vi "Backpressure test CIF Pcap.vi"() -> ()   [LabVIEW 2021]
uses:
  Iceoryx.lvlib
  typedef/CIF Pcap Publisher Configuration.ctl
  typedef/CIF Pcap Subscriber Configuration.ctl
  typedef/CIF Channel Header Publisher.ctl
panel:
  out "status":string
  out "pass":bool
  out "error out":errorcluster
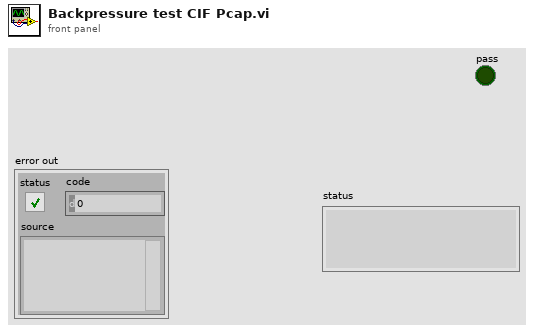
[diagram p1: front panel]
types:
  T1 = typedef "Iceoryx.lvlib/CIF Pcap Subscriber Configuration.ctl" = cluster{"Name":string, "Topic":string, "Link Type":u32, "Backpressure":bool}
  T2 = typedef "Iceoryx.lvlib/CIF Pcap Publisher Configuration.ctl" = cluster{"Name":string, "Topic":string, "Link Type":u32, "Descriptor":string, "Max Bytes":u32, "Best Effort Subscribers":u32, "Backpressure Subscribers":u32, "Best Effort Queue Depth":u32, "Backpressure Queue Depth":u32}
  T3 = typedef "Iceoryx.lvlib/CIF Channel Header Publisher.ctl" = cluster{"T0":i64, "T_Out":i64, "T_Tx":i64, "ClockID":u8}
  T4 = typedef "Iceoryx.lvlib/CIF Publisher Refnum.ctl" = cluster{"refnum":u64, "CIF Pub":enum8{"cifpub"}}
  T5 = typedef "Iceoryx.lvlib/CIF Subscriber Refnum.ctl" = cluster{"refnum":u64, "CIF Sub":enum8{"cifsub"}}
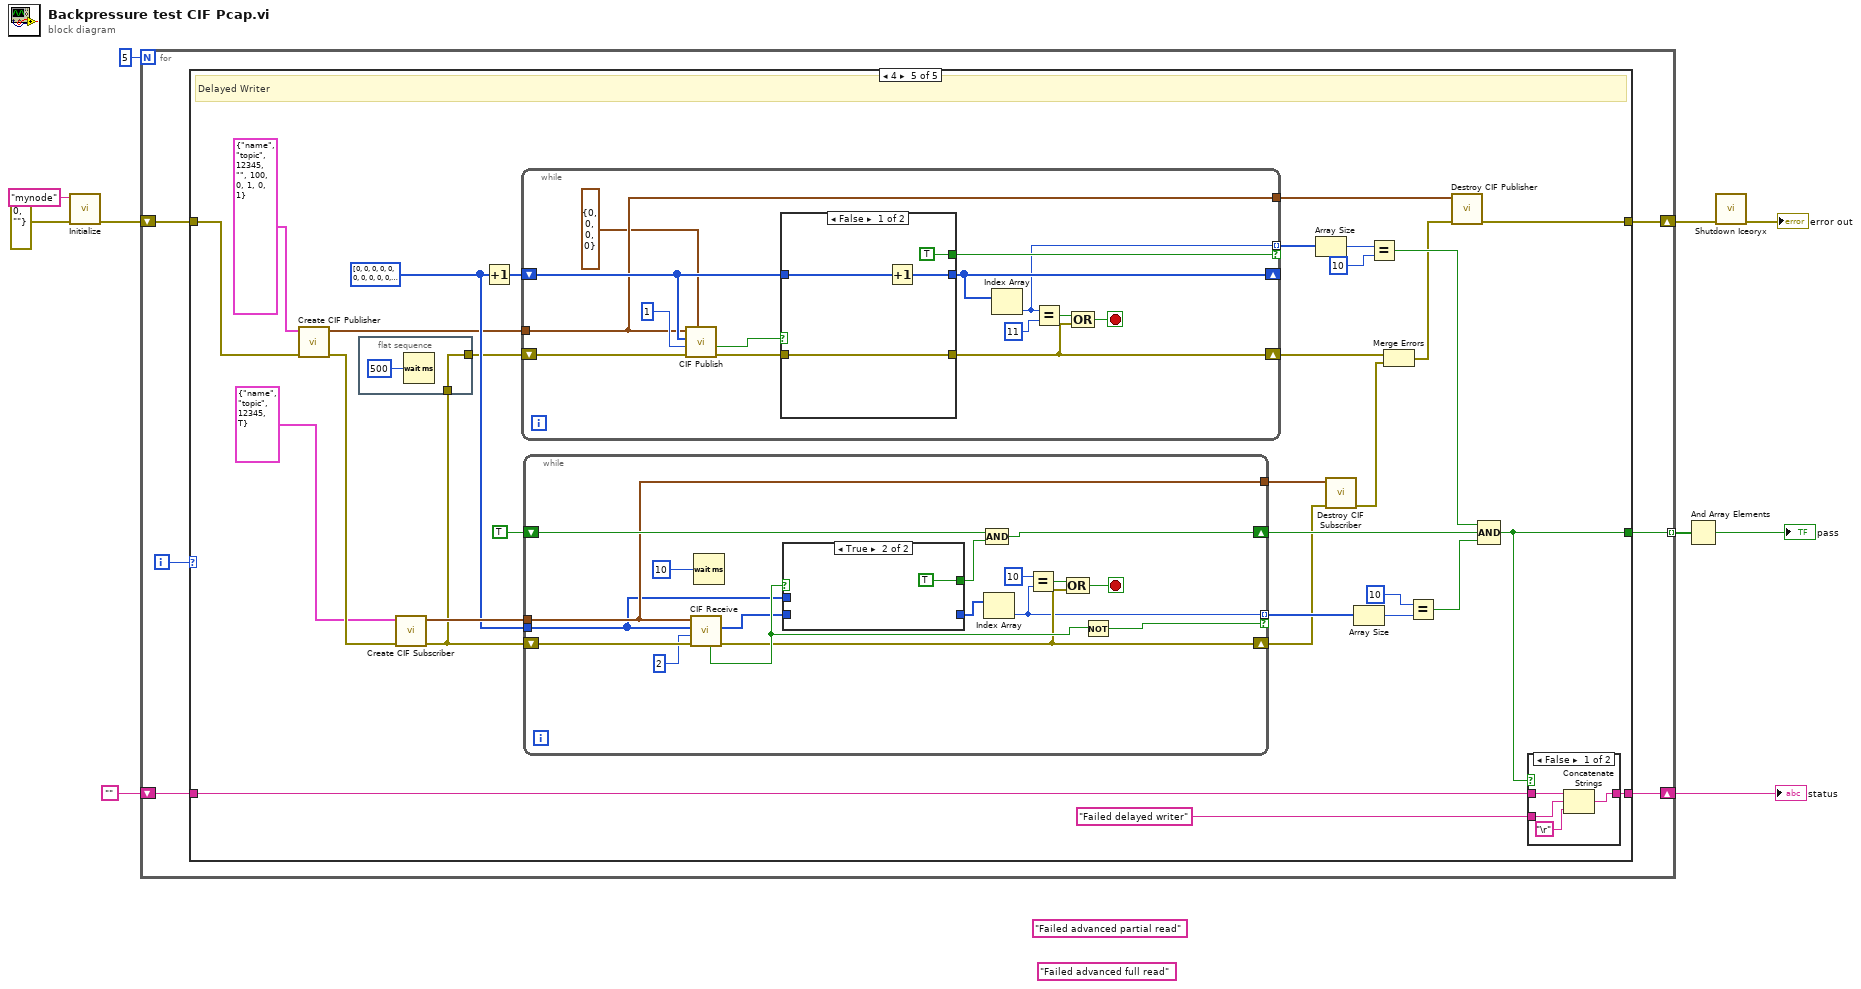
[diagram p0: block diagram]
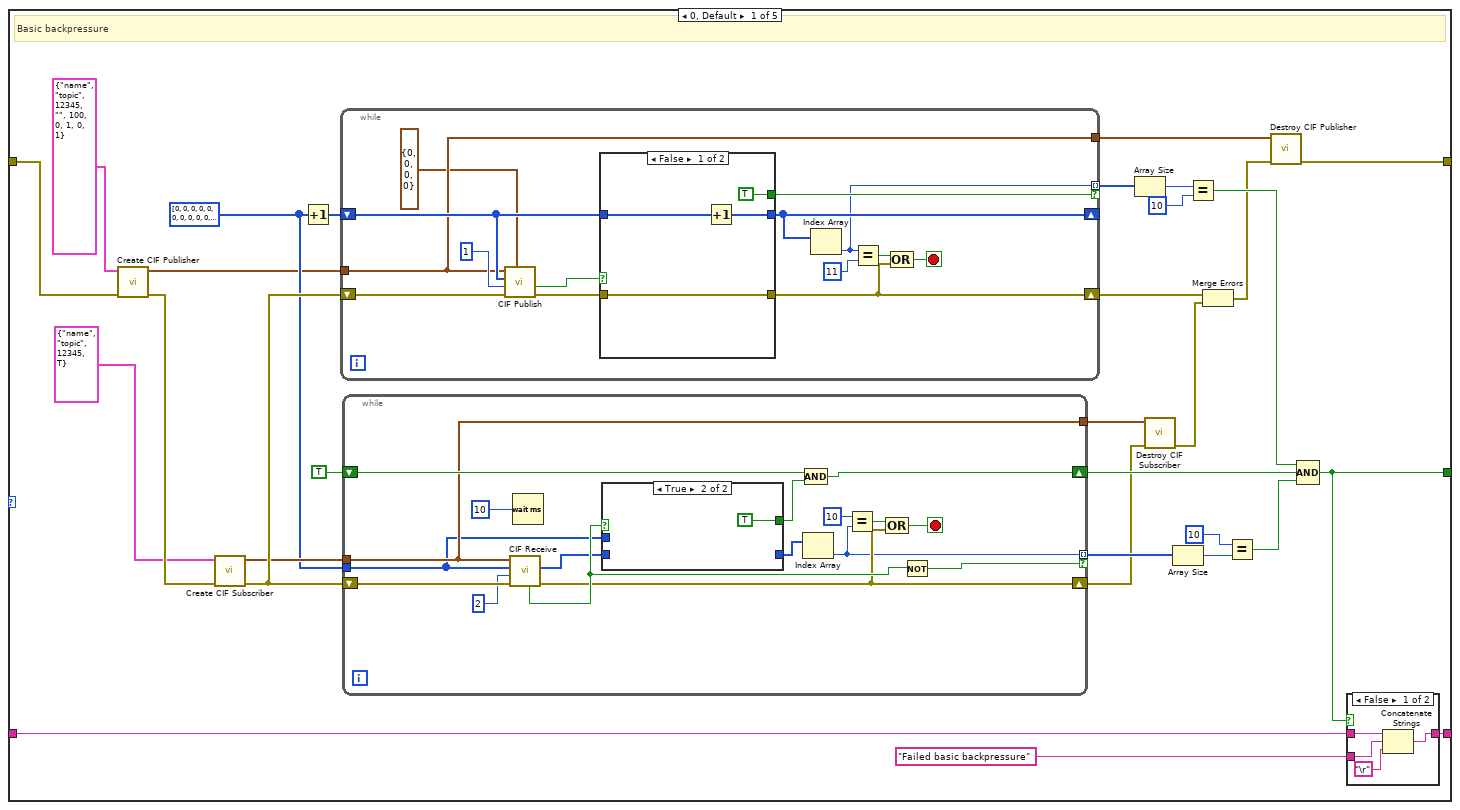
[diagram p2: hidden frame]
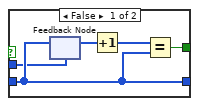
[diagram p3: hidden frame]
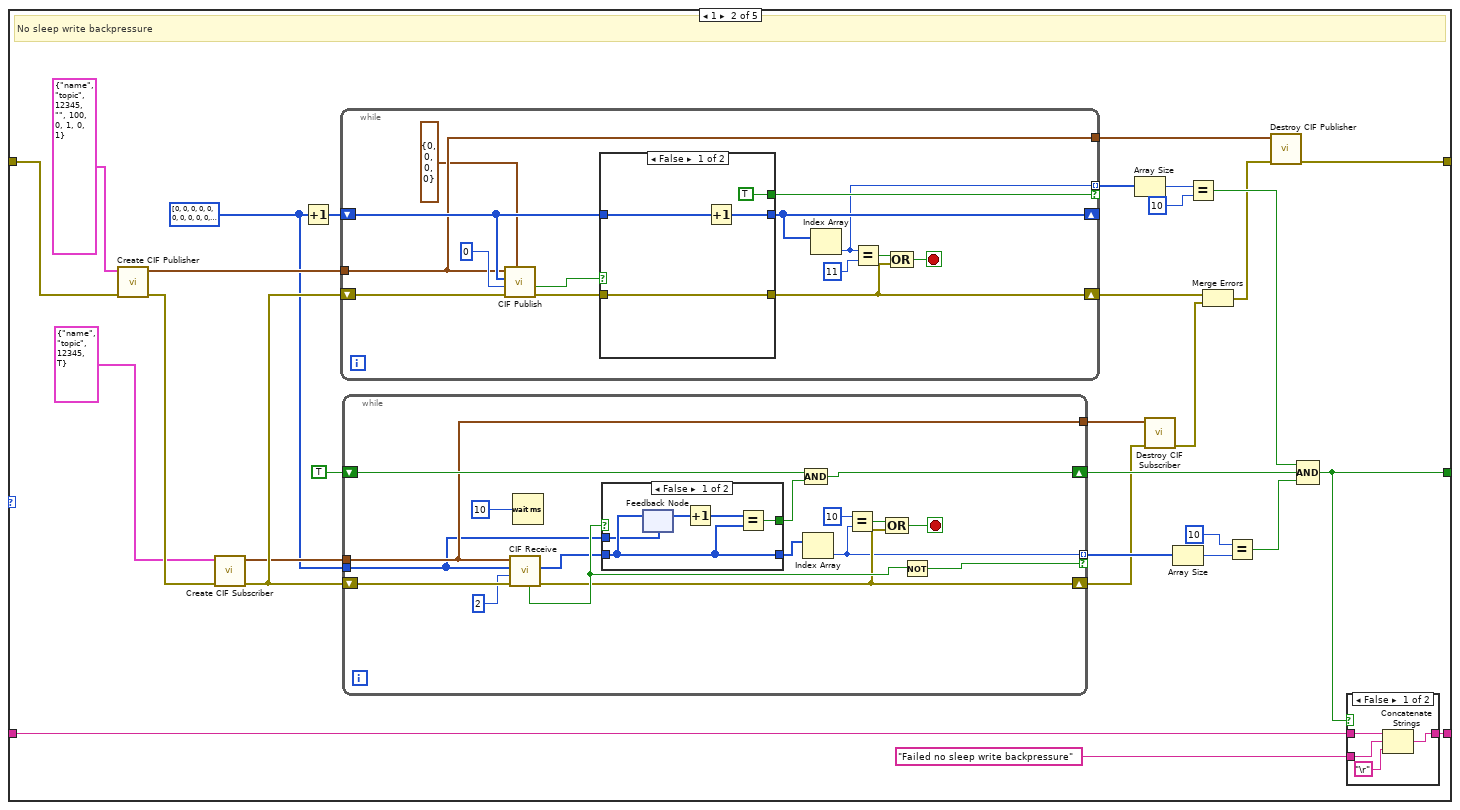
[diagram p6: hidden frame]
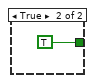
[diagram p7: hidden frame]
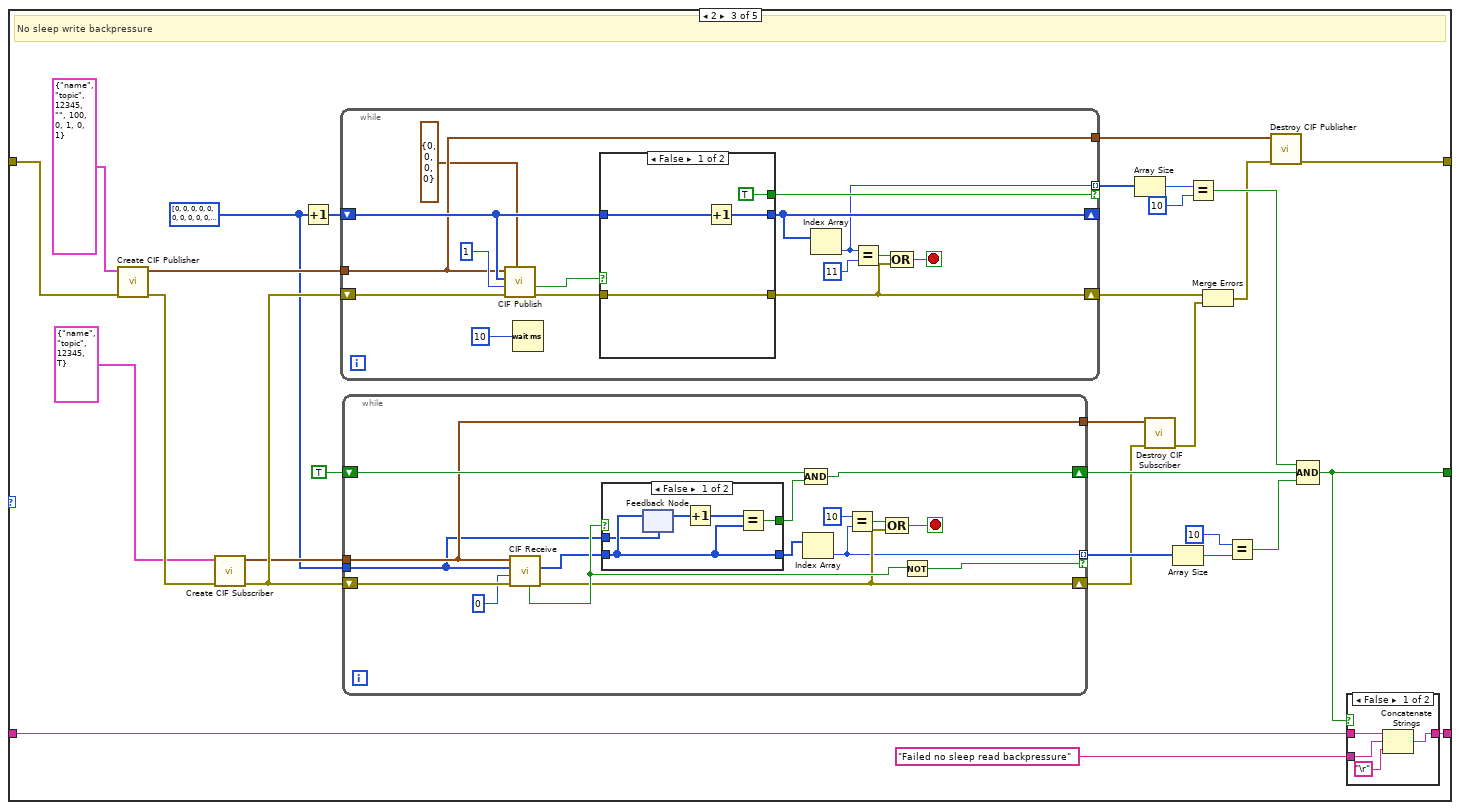
[diagram p10: hidden frame]
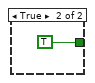
[diagram p11: hidden frame]
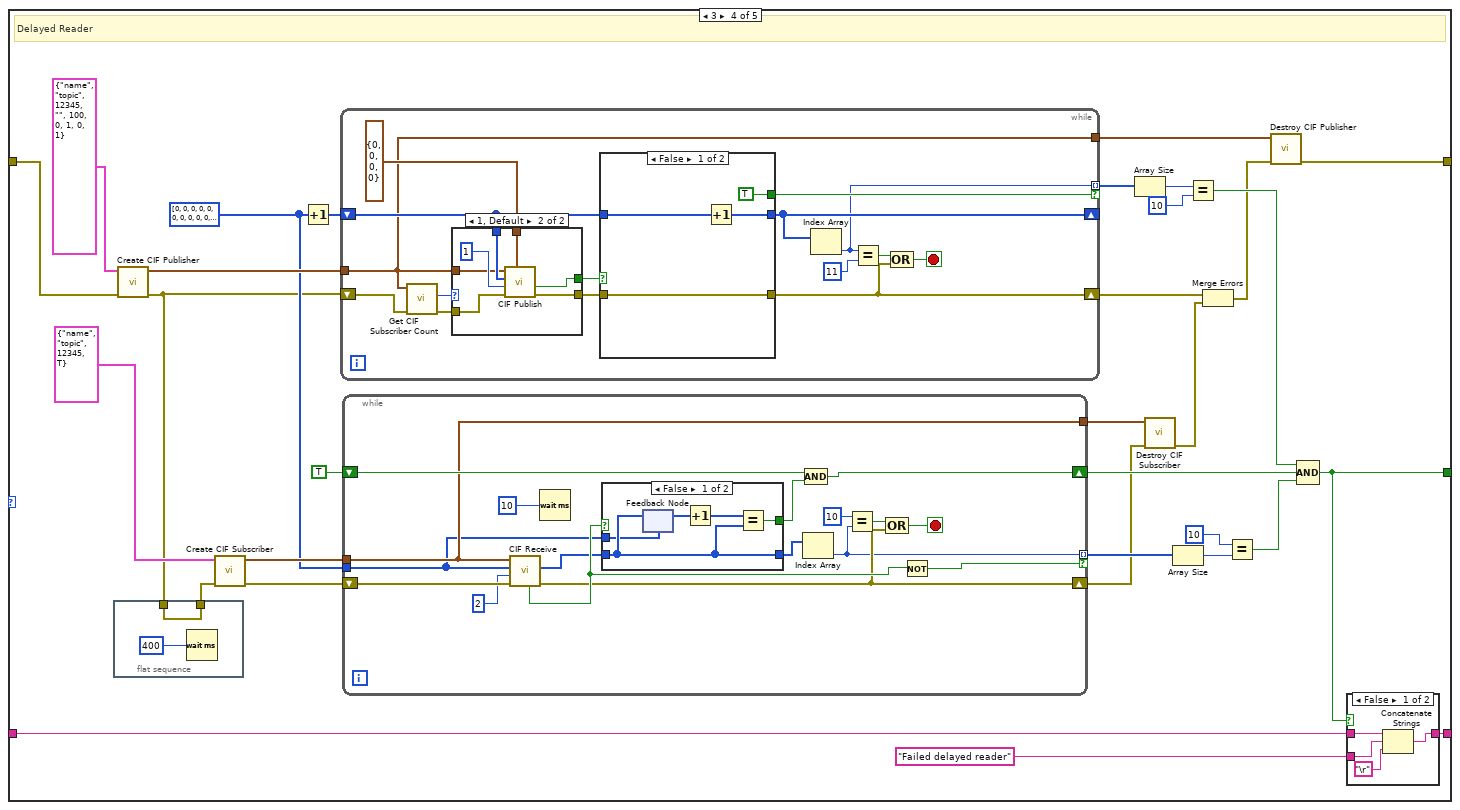
[diagram p14: hidden frame]
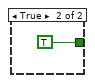
[diagram p15: hidden frame]
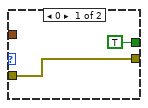
[diagram p16: hidden frame]
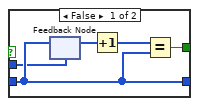
[diagram p19: hidden frame]
diagram:
  (unwired) "Failed advanced partial read"
  (unwired) "Failed advanced full read"
  n1 = call "Initialize.vi"("error in (no error)"=errorcluster {"status"=FALSE, "code"=0, "source"=""} ("error out"), "Node name"="mynode") -> ("error out"=w4:errorcluster)  [unwired: 9 in]
  n2 = for {
    N: 5 -> [_]
    tunnel: [w16] -> w10 mode=indexing
    shift-right: [w13] -> w6
    shift-left: "" -> [w14]
    shift-right: [w12] -> w2
    shift-left: w4 -> [w11]
    i -> [w15]
    n3 = case shown="4" w15 {
      tunnel: [w36 w114 w192 w271 w362] -> w16
      tunnel: w14 -> [w46 w124 w202 w281 w372]
      tunnel: [w45 w123 w201 w280 w371] -> w13
      tunnel: [w20 w97 w175 w256 w347] -> w12
      tunnel: w11 -> [w31 w109 w187 w266 w357]
      frame 0, Default {
        w19 = u8[] [0, 0, 0, 0, 0, 0, 0, 0, 0, 0, 0, 0, 0, 0, 0, 0, 0, 0, 0, 0, 0, 0, 0, 0, 0, 0, 0, 0, 0, 0, 0, 0, 0, 0, 0, 0, 0, 0, 0, 0, 0, 0, 0, 0, 0, 0, 0, 0, 0, 0, 0, 0, 0, 0, 0, 0, 0, 0, 0, 0, 0, 0, 0, 0, 0, 0, 0, 0, 0, 0, 0, 0, 0, 0, 0, 0, 0, 0, 0, 0, 0, 0, 0, 0, 0, 0, 0, 0, 0, 0, 0, 0, 0, 0, 0, 0, 0, 0, 0, 0] ("Data In")
        # "Basic backpressure"
        n4 = call "Create CIF Publisher.vi"("error in (no error)"=w31, "CIF Pcap Publisher Configuration"=T2 {"Name"="name", "Topic"="topic", "Link Type"=12345, "Descriptor"="", "Max Bytes"=100, "Best Effort Subscribers"=0, "Backpressure Subscribers"=1, "Best Effort Queue Depth"=0, "Backpressure Queue Depth"=1}) -> ("error out"=w29:errorcluster, "CIF Publisher Refnum"=w17:T4)  [unwired: 8 in]
        n5 = call "Create CIF Subscriber.vi"("error in (no error)"=w29, "CIF Pcap Subscriber Configuration"=T1 {"Name"="name", "Topic"="topic", "Link Type"=12345, "Backpressure"=TRUE}) -> ("error out"=w27:errorcluster, "CIF Subscriber Refnum"=w26:T5)  [unwired: 8 in]
        n6 = Increment(x=w19) -> (x+1=w18:u8[])
        n7 = while {
          tunnel: w17 -> [w73]
          shift-right: [w81] -> w43
          shift-left: w27 -> [w78]
          shift-right: [w72] -> _
          shift-left: w18 -> [w74]
          tunnel: [w71] -> w35 mode=indexing if=w79
          tunnel: [w73] -> w22
          stop <- w80 stop-if-true
          n8 = call "CIF Publish.vi"("CIF Channel Header Publisher"=T3 {"T0"=0, "T_Out"=0, "T_Tx"=0, "ClockID"=0}, "error in (no error)"=w78, "Timeout ms"=u32 1 ("Timoeut ms"), "Data In"=w74, "Publisher Reference"=w73) -> ("error out"=w77:errorcluster, "Timeout"=w76:bool)  [unwired: 3 in, 2 out]
          n9 = case shown="False" w76 {
            tunnel: w77 -> [w84 w89]
            tunnel: [w84 w89] -> w81
            tunnel: w74 -> [w87 w88]
            tunnel: [w86 w88] -> w72
            tunnel: [TRUE _] -> w79
            frame False {
              n10 = Increment(x=w87) -> (x+1=w86:u8[])
            }
            frame True {
              # "Timeout"
            }
          }
          n11 = Index Array(array=w72) -> (element=w71:u8)  [unwired: 1 in]
          n12 = Equal?(x=w71, y=u8 11) -> (x = y?=w82:bool)
          n13 = Compound Arithmetic op=OR(w82, w81) -> (w80:bool)
        }
        n14 = while {
          shift-right: [w60] -> w38
          shift-left: TRUE -> [w62]
          shift-right: [w50] -> w24
          shift-left: w27 -> [w55]
          tunnel: [w47] -> w41 mode=indexing if=w56
          tunnel: w26 -> [w53]
          tunnel: [w53] -> w25
          tunnel: w19 -> [w49]
          stop <- w57 stop-if-true
          n15 = call "CIF Receive.vi"("error in (no error)"=w55, "Timoeut ms"=u32 2, "Data In"=w49, "Subscriber Reference"=w53) -> ("error out"=w50:errorcluster, "Data Out"=w51:u8[], "Timeout"=w54:bool)  [unwired: 2 in, 3 out]
          n16 = Wait (ms)(milliseconds to wait=u32 10) -> ()  [unwired: 1 out]
          n17 = case shown="True" w54 {
            tunnel: w51 -> [w65 _]
            tunnel: [w66 TRUE] -> w61
            tunnel: [w65 _] -> w48
            tunnel: w49 -> [w64 _]
            frame False {
              n18 = feedback #1(w64) -> (w68:u8[])
              n19 = feedback-in #1(w65) -> ()
              n20 = Increment(x=w68) -> (x+1=w67:u8[])
              n21 = Equal?(x=w67, y=w65) -> (x = y?=w66:bool)
            }
            frame True {
            }
          }
          n22 = Index Array(array=w48) -> (element=w47:u8)  [unwired: 1 in]
          n23 = Compound Arithmetic op=AND(w62, w61) -> (w60:bool)
          n24 = Equal?(x=u8 10, y=w47) -> (x = y?=w58:bool)
          n25 = Compound Arithmetic op=OR(w58, w50) -> (w57:bool)
          n26 = Not(x=w54) -> (.not. x?=w56:bool)
        }
        n27 = Array Size(array=w35) -> (size(s)=w34:i32)
        n28 = call "Destroy CIF Subscriber.vi"("error in (no error)"=w24, "Subscriber Reference"=w25) -> ("error out"=w23:errorcluster)  [unwired: 9 in]
        n29 = Array Size(array=w41) -> (size(s)=w40:i32)
        n30 = Equal?(x=w34, y=10 ("x")) -> (x = y?=w32:bool)
        n31 = Merge Errors(w43, w23) -> (w21:errorcluster)
        n32 = Equal?(x=10, y=w40) -> (x = y?=w37:bool)
        n33 = call "Destroy CIF Publisher.vi"("error in (no error)"=w21, "Publisher Reference"=w22) -> ("error out"=w20:errorcluster)  [unwired: 9 in]
        n34 = Compound Arithmetic op=AND(w32, w38, w37) -> (w36:bool)
        n35 = case shown="False" w36 {
          tunnel: w46 -> [w93 w94]
          tunnel: [w91 w94] -> w45
          tunnel: "Failed basic backpressure" -> [w92 _]
          frame False {
            n36 = Concatenate Strings(w93, w92, "\r") -> (w91:string)
          }
          frame True {
          }
        }
      }
      frame 1 {
        w96 = u8[] [0, 0, 0, 0, 0, 0, 0, 0, 0, 0, 0, 0, 0, 0, 0, 0, 0, 0, 0, 0, 0, 0, 0, 0, 0, 0, 0, 0, 0, 0, 0, 0, 0, 0, 0, 0, 0, 0, 0, 0, 0, 0, 0, 0, 0, 0, 0, 0, 0, 0, 0, 0, 0, 0, 0, 0, 0, 0, 0, 0, 0, 0, 0, 0, 0, 0, 0, 0, 0, 0, 0, 0, 0, 0, 0, 0, 0, 0, 0, 0, 0, 0, 0, 0, 0, 0, 0, 0, 0, 0, 0, 0, 0, 0, 0, 0, 0, 0, 0, 0] ("Data In")
        # "No sleep write backpressure"
        n37 = call "Create CIF Publisher.vi"("error in (no error)"=w109, "CIF Pcap Publisher Configuration"=T2 {"Name"="name", "Topic"="topic", "Link Type"=12345, "Descriptor"="", "Max Bytes"=100, "Best Effort Subscribers"=0, "Backpressure Subscribers"=1, "Best Effort Queue Depth"=0, "Backpressure Queue Depth"=1}) -> ("error out"=w106:errorcluster, "CIF Publisher Refnum"=w107:T4)  [unwired: 8 in]
        n38 = call "Create CIF Subscriber.vi"("error in (no error)"=w106, "CIF Pcap Subscriber Configuration"=T1 {"Name"="name", "Topic"="topic", "Link Type"=12345, "Backpressure"=TRUE}) -> ("error out"=w104:errorcluster, "CIF Subscriber Refnum"=w103:T5)  [unwired: 8 in]
        n39 = Increment(x=w96) -> (x+1=w95:u8[])
        n40 = while {
          tunnel: w107 -> [w151]
          shift-right: [w159] -> w121
          shift-left: w104 -> [w156]
          shift-right: [w150] -> _
          shift-left: w95 -> [w152]
          tunnel: [w149] -> w113 mode=indexing if=w157
          tunnel: [w151] -> w99
          stop <- w158 stop-if-true
          n41 = call "CIF Publish.vi"("CIF Channel Header Publisher"=T3 {"T0"=0, "T_Out"=0, "T_Tx"=0, "ClockID"=0}, "error in (no error)"=w156, "Timeout ms"=u32 0 ("Timoeut ms"), "Data In"=w152, "Publisher Reference"=w151) -> ("error out"=w155:errorcluster, "Timeout"=w154:bool)  [unwired: 3 in, 2 out]
          n42 = case shown="False" w154 {
            tunnel: w155 -> [w162 w167]
            tunnel: [w162 w167] -> w159
            tunnel: w152 -> [w165 w166]
            tunnel: [w164 w166] -> w150
            tunnel: [TRUE _] -> w157
            frame False {
              n43 = Increment(x=w165) -> (x+1=w164:u8[])
            }
            frame True {
              # "Timeout"
            }
          }
          n44 = Index Array(array=w150) -> (element=w149:u8)  [unwired: 1 in]
          n45 = Equal?(x=w149, y=u8 11) -> (x = y?=w160:bool)
          n46 = Compound Arithmetic op=OR(w160, w159) -> (w158:bool)
        }
        n47 = while {
          shift-right: [w138] -> w116
          shift-left: TRUE -> [w140]
          shift-right: [w128] -> w101
          shift-left: w104 -> [w133]
          tunnel: [w125] -> w119 mode=indexing if=w134
          tunnel: w103 -> [w131]
          tunnel: [w131] -> w102
          tunnel: w96 -> [w127]
          stop <- w135 stop-if-true
          n48 = call "CIF Receive.vi"("error in (no error)"=w133, "Timoeut ms"=u32 2, "Data In"=w127, "Subscriber Reference"=w131) -> ("error out"=w128:errorcluster, "Data Out"=w129:u8[], "Timeout"=w132:bool)  [unwired: 2 in, 3 out]
          n49 = Wait (ms)(milliseconds to wait=u32 10) -> ()  [unwired: 1 out]
          n50 = case shown="False" w132 {
            tunnel: w129 -> [w143 _]
            tunnel: [w144 TRUE] -> w139
            tunnel: [w143 _] -> w126
            tunnel: w127 -> [w142 _]
            frame False {
              n51 = feedback #2(w142) -> (w146:u8[])
              n52 = feedback-in #2(w143) -> ()
              n53 = Increment(x=w146) -> (x+1=w145:u8[])
              n54 = Equal?(x=w145, y=w143) -> (x = y?=w144:bool)
            }
            frame True {
            }
          }
          n55 = Index Array(array=w126) -> (element=w125:u8)  [unwired: 1 in]
          n56 = Compound Arithmetic op=AND(w140, w139) -> (w138:bool)
          n57 = Equal?(x=u8 10, y=w125) -> (x = y?=w136:bool)
          n58 = Compound Arithmetic op=OR(w136, w128) -> (w135:bool)
          n59 = Not(x=w132) -> (.not. x?=w134:bool)
        }
        n60 = Array Size(array=w113) -> (size(s)=w112:i32)
        n61 = call "Destroy CIF Subscriber.vi"("error in (no error)"=w101, "Subscriber Reference"=w102) -> ("error out"=w100:errorcluster)  [unwired: 9 in]
        n62 = Array Size(array=w119) -> (size(s)=w118:i32)
        n63 = Equal?(x=w112, y=10 ("x")) -> (x = y?=w110:bool)
        n64 = Merge Errors(w121, w100) -> (w98:errorcluster)
        n65 = Equal?(x=10, y=w118) -> (x = y?=w115:bool)
        n66 = call "Destroy CIF Publisher.vi"("error in (no error)"=w98, "Publisher Reference"=w99) -> ("error out"=w97:errorcluster)  [unwired: 9 in]
        n67 = Compound Arithmetic op=AND(w110, w116, w115) -> (w114:bool)
        n68 = case shown="False" w114 {
          tunnel: w124 -> [w171 w172]
          tunnel: [w169 w172] -> w123
          tunnel: "Failed no sleep write backpressure" -> [w170 _]
          frame False {
            n69 = Concatenate Strings(w171, w170, "\r") -> (w169:string)
          }
          frame True {
          }
        }
      }
      frame 2 {
        w174 = u8[] [0, 0, 0, 0, 0, 0, 0, 0, 0, 0, 0, 0, 0, 0, 0, 0, 0, 0, 0, 0, 0, 0, 0, 0, 0, 0, 0, 0, 0, 0, 0, 0, 0, 0, 0, 0, 0, 0, 0, 0, 0, 0, 0, 0, 0, 0, 0, 0, 0, 0, 0, 0, 0, 0, 0, 0, 0, 0, 0, 0, 0, 0, 0, 0, 0, 0, 0, 0, 0, 0, 0, 0, 0, 0, 0, 0, 0, 0, 0, 0, 0, 0, 0, 0, 0, 0, 0, 0, 0, 0, 0, 0, 0, 0, 0, 0, 0, 0, 0, 0] ("Data In")
        # "No sleep write backpressure"
        n70 = call "Create CIF Publisher.vi"("error in (no error)"=w187, "CIF Pcap Publisher Configuration"=T2 {"Name"="name", "Topic"="topic", "Link Type"=12345, "Descriptor"="", "Max Bytes"=100, "Best Effort Subscribers"=0, "Backpressure Subscribers"=1, "Best Effort Queue Depth"=0, "Backpressure Queue Depth"=1}) -> ("error out"=w184:errorcluster, "CIF Publisher Refnum"=w185:T4)  [unwired: 8 in]
        n71 = call "Create CIF Subscriber.vi"("error in (no error)"=w184, "CIF Pcap Subscriber Configuration"=T1 {"Name"="name", "Topic"="topic", "Link Type"=12345, "Backpressure"=TRUE}) -> ("error out"=w182:errorcluster, "CIF Subscriber Refnum"=w181:T5)  [unwired: 8 in]
        n72 = Increment(x=w174) -> (x+1=w173:u8[])
        n73 = while {
          tunnel: w185 -> [w229]
          shift-right: [w237] -> w199
          shift-left: w182 -> [w234]
          shift-right: [w228] -> _
          shift-left: w173 -> [w230]
          tunnel: [w227] -> w191 mode=indexing if=w235
          tunnel: [w229] -> w177
          stop <- w236 stop-if-true
          n74 = call "CIF Publish.vi"("CIF Channel Header Publisher"=T3 {"T0"=0, "T_Out"=0, "T_Tx"=0, "ClockID"=0}, "error in (no error)"=w234, "Timeout ms"=u32 1 ("Timoeut ms"), "Data In"=w230, "Publisher Reference"=w229) -> ("error out"=w233:errorcluster, "Timeout"=w232:bool)  [unwired: 3 in, 2 out]
          n75 = Wait (ms)(milliseconds to wait=u32 10) -> ()  [unwired: 1 out]
          n76 = case shown="False" w232 {
            tunnel: w233 -> [w240 w245]
            tunnel: [w240 w245] -> w237
            tunnel: w230 -> [w243 w244]
            tunnel: [w242 w244] -> w228
            tunnel: [TRUE _] -> w235
            frame False {
              n77 = Increment(x=w243) -> (x+1=w242:u8[])
            }
            frame True {
              # "Timeout"
            }
          }
          n78 = Index Array(array=w228) -> (element=w227:u8)  [unwired: 1 in]
          n79 = Equal?(x=w227, y=u8 11) -> (x = y?=w238:bool)
          n80 = Compound Arithmetic op=OR(w238, w237) -> (w236:bool)
        }
        n81 = while {
          shift-right: [w216] -> w194
          shift-left: TRUE -> [w218]
          shift-right: [w206] -> w179
          shift-left: w182 -> [w211]
          tunnel: [w203] -> w197 mode=indexing if=w212
          tunnel: w181 -> [w209]
          tunnel: [w209] -> w180
          tunnel: w174 -> [w205]
          stop <- w213 stop-if-true
          n82 = call "CIF Receive.vi"("error in (no error)"=w211, "Timoeut ms"=u32 0, "Data In"=w205, "Subscriber Reference"=w209) -> ("error out"=w206:errorcluster, "Data Out"=w207:u8[], "Timeout"=w210:bool)  [unwired: 2 in, 3 out]
          n83 = case shown="False" w210 {
            tunnel: w207 -> [w220 _]
            tunnel: [w221 TRUE] -> w217
            tunnel: [w220 _] -> w204
            tunnel: w205 -> [w219 _]
            frame False {
              n84 = feedback #3(w219) -> (w223:u8[])
              n85 = feedback-in #3(w220) -> ()
              n86 = Increment(x=w223) -> (x+1=w222:u8[])
              n87 = Equal?(x=w222, y=w220) -> (x = y?=w221:bool)
            }
            frame True {
            }
          }
          n88 = Index Array(array=w204) -> (element=w203:u8)  [unwired: 1 in]
          n89 = Compound Arithmetic op=AND(w218, w217) -> (w216:bool)
          n90 = Equal?(x=u8 10, y=w203) -> (x = y?=w214:bool)
          n91 = Compound Arithmetic op=OR(w214, w206) -> (w213:bool)
          n92 = Not(x=w210) -> (.not. x?=w212:bool)
        }
        n93 = Array Size(array=w191) -> (size(s)=w190:i32)
        n94 = call "Destroy CIF Subscriber.vi"("error in (no error)"=w179, "Subscriber Reference"=w180) -> ("error out"=w178:errorcluster)  [unwired: 9 in]
        n95 = Array Size(array=w197) -> (size(s)=w196:i32)
        n96 = Equal?(x=w190, y=10 ("x")) -> (x = y?=w188:bool)
        n97 = Merge Errors(w199, w178) -> (w176:errorcluster)
        n98 = Equal?(x=10, y=w196) -> (x = y?=w193:bool)
        n99 = call "Destroy CIF Publisher.vi"("error in (no error)"=w176, "Publisher Reference"=w177) -> ("error out"=w175:errorcluster)  [unwired: 9 in]
        n100 = Compound Arithmetic op=AND(w188, w194, w193) -> (w192:bool)
        n101 = case shown="False" w192 {
          tunnel: w202 -> [w249 w250]
          tunnel: [w247 w250] -> w201
          tunnel: "Failed no sleep read backpressure" -> [w248 _]
          frame False {
            n102 = Concatenate Strings(w249, w248, "\r") -> (w247:string)
          }
          frame True {
          }
        }
      }
      frame 3 {
        w255 = u8[] [0, 0, 0, 0, 0, 0, 0, 0, 0, 0, 0, 0, 0, 0, 0, 0, 0, 0, 0, 0, 0, 0, 0, 0, 0, 0, 0, 0, 0, 0, 0, 0, 0, 0, 0, 0, 0, 0, 0, 0, 0, 0, 0, 0, 0, 0, 0, 0, 0, 0, 0, 0, 0, 0, 0, 0, 0, 0, 0, 0, 0, 0, 0, 0, 0, 0, 0, 0, 0, 0, 0, 0, 0, 0, 0, 0, 0, 0, 0, 0, 0, 0, 0, 0, 0, 0, 0, 0, 0, 0, 0, 0, 0, 0, 0, 0, 0, 0, 0, 0] ("Data In")
        # "Delayed Reader"
        n103 = flat-sequence {
          tunnel: w251 -> [w283]
          tunnel: [w283] -> w253
          frame #0 {
            n104 = Wait (ms)(milliseconds to wait=u32 400) -> ()  [unwired: 1 out]
          }
        }
        n105 = call "Create CIF Publisher.vi"("error in (no error)"=w266, "CIF Pcap Publisher Configuration"=T2 {"Name"="name", "Topic"="topic", "Link Type"=12345, "Descriptor"="", "Max Bytes"=100, "Best Effort Subscribers"=0, "Backpressure Subscribers"=1, "Best Effort Queue Depth"=0, "Backpressure Queue Depth"=1}) -> ("error out"=w251:errorcluster, "CIF Publisher Refnum"=w264:T4)  [unwired: 8 in]
        n106 = call "Create CIF Subscriber.vi"("error in (no error)"=w253, "CIF Pcap Subscriber Configuration"=T1 {"Name"="name", "Topic"="topic", "Link Type"=12345, "Backpressure"=TRUE}) -> ("error out"=w252:errorcluster, "CIF Subscriber Refnum"=w262:T5)  [unwired: 8 in]
        n107 = Increment(x=w255) -> (x+1=w254:u8[])
        n108 = while {
          tunnel: w264 -> [w307]
          shift-right: [w319] -> w278
          shift-left: w251 -> [w310]
          shift-right: [w313] -> _
          shift-left: w254 -> [w314]
          tunnel: [w312] -> w270 mode=indexing if=w317
          tunnel: [w307] -> w258
          stop <- w318 stop-if-true
          n109 = call "Get CIF Subscriber Count.vi"("error in (no error)"=w310, "Publisher Reference"=w307) -> ("error out"=w309:errorcluster, "Backpressure"=w308:u32)  [unwired: 7 in, 1 out]
          n110 = case shown="1, Default" w308 {
            tunnel: [w323 w330] -> w316
            tunnel: [TRUE ("Timeout") w329] -> w315
            tunnel: w314 -> [_ w327]
            tunnel: T3 {"T0"=0, "T_Out"=0, "T_Tx"=0, "ClockID"=0} ("CIF Channel Header Publisher") -> [_ w326]
            tunnel: w307 -> [_ w325]
            tunnel: w309 -> [w323 w324]
            frame 0 {
            }
            frame 1, Default {
              n111 = call "CIF Publish.vi"("CIF Channel Header Publisher"=w326, "error in (no error)"=w324, "Timeout ms"=u32 1 ("Timoeut ms"), "Data In"=w327, "Publisher Reference"=w325) -> ("error out"=w330:errorcluster, "Timeout"=w329:bool)  [unwired: 3 in, 2 out]
            }
          }
          n112 = case shown="False" w315 {
            tunnel: w316 -> [w331 w336]
            tunnel: [w331 w336] -> w319
            tunnel: w314 -> [w334 w335]
            tunnel: [w333 w335] -> w313
            tunnel: [TRUE _] -> w317
            frame False {
              n113 = Increment(x=w334) -> (x+1=w333:u8[])
            }
            frame True {
              # "Timeout"
            }
          }
          n114 = Index Array(array=w313) -> (element=w312:u8)  [unwired: 1 in]
          n115 = Equal?(x=w312, y=u8 11) -> (x = y?=w320:bool)
          n116 = Compound Arithmetic op=OR(w320, w319) -> (w318:bool)
        }
        n117 = while {
          shift-right: [w298] -> w273
          shift-left: TRUE -> [w300]
          shift-right: [w288] -> w260
          shift-left: w252 -> [w293]
          tunnel: [w285] -> w276 mode=indexing if=w294
          tunnel: w262 -> [w291]
          tunnel: [w291] -> w261
          tunnel: w255 -> [w287]
          stop <- w295 stop-if-true
          n118 = call "CIF Receive.vi"("error in (no error)"=w293, "Timoeut ms"=u32 2, "Data In"=w287, "Subscriber Reference"=w291) -> ("error out"=w288:errorcluster, "Data Out"=w289:u8[], "Timeout"=w292:bool)  [unwired: 2 in, 3 out]
          n119 = Wait (ms)(milliseconds to wait=u32 10) -> ()  [unwired: 1 out]
          n120 = case shown="False" w292 {
            tunnel: w289 -> [w302 _]
            tunnel: [w303 TRUE] -> w299
            tunnel: [w302 _] -> w286
            tunnel: w287 -> [w301 _]
            frame False {
              n121 = feedback #4(w301) -> (w305:u8[])
              n122 = feedback-in #4(w302) -> ()
              n123 = Increment(x=w305) -> (x+1=w304:u8[])
              n124 = Equal?(x=w304, y=w302) -> (x = y?=w303:bool)
            }
            frame True {
            }
          }
          n125 = Index Array(array=w286) -> (element=w285:u8)  [unwired: 1 in]
          n126 = Compound Arithmetic op=AND(w300, w299) -> (w298:bool)
          n127 = Equal?(x=u8 10, y=w285) -> (x = y?=w296:bool)
          n128 = Compound Arithmetic op=OR(w296, w288) -> (w295:bool)
          n129 = Not(x=w292) -> (.not. x?=w294:bool)
        }
        n130 = Array Size(array=w270) -> (size(s)=w269:i32)
        n131 = call "Destroy CIF Subscriber.vi"("error in (no error)"=w260, "Subscriber Reference"=w261) -> ("error out"=w259:errorcluster)  [unwired: 9 in]
        n132 = Array Size(array=w276) -> (size(s)=w275:i32)
        n133 = Equal?(x=w269, y=10 ("x")) -> (x = y?=w267:bool)
        n134 = Merge Errors(w278, w259) -> (w257:errorcluster)
        n135 = Equal?(x=10, y=w275) -> (x = y?=w272:bool)
        n136 = call "Destroy CIF Publisher.vi"("error in (no error)"=w257, "Publisher Reference"=w258) -> ("error out"=w256:errorcluster)  [unwired: 9 in]
        n137 = Compound Arithmetic op=AND(w267, w273, w272) -> (w271:bool)
        n138 = case shown="False" w271 {
          tunnel: w281 -> [w340 w341]
          tunnel: [w338 w341] -> w280
          tunnel: "Failed delayed reader" -> [w339 _]
          frame False {
            n139 = Concatenate Strings(w340, w339, "\r") -> (w338:string)
          }
          frame True {
          }
        }
      }
      frame 4 {
        w346 = u8[] [0, 0, 0, 0, 0, 0, 0, 0, 0, 0, 0, 0, 0, 0, 0, 0, 0, 0, 0, 0, 0, 0, 0, 0, 0, 0, 0, 0, 0, 0, 0, 0, 0, 0, 0, 0, 0, 0, 0, 0, 0, 0, 0, 0, 0, 0, 0, 0, 0, 0, 0, 0, 0, 0, 0, 0, 0, 0, 0, 0, 0, 0, 0, 0, 0, 0, 0, 0, 0, 0, 0, 0, 0, 0, 0, 0, 0, 0, 0, 0, 0, 0, 0, 0, 0, 0, 0, 0, 0, 0, 0, 0, 0, 0, 0, 0, 0, 0, 0, 0] ("Data In")
        # "Delayed Writer"
        n140 = call "Create CIF Publisher.vi"("error in (no error)"=w357, "CIF Pcap Publisher Configuration"=T2 {"Name"="name", "Topic"="topic", "Link Type"=12345, "Descriptor"="", "Max Bytes"=100, "Best Effort Subscribers"=0, "Backpressure Subscribers"=1, "Best Effort Queue Depth"=0, "Backpressure Queue Depth"=1}) -> ("error out"=w355:errorcluster, "CIF Publisher Refnum"=w344:T4)  [unwired: 8 in]
        n141 = flat-sequence {
          tunnel: [w373] -> w342
          tunnel: w343 -> [w373]
          frame #0 {
            n142 = Wait (ms)(milliseconds to wait=u32 500) -> ()  [unwired: 1 out]
          }
        }
        n143 = call "Create CIF Subscriber.vi"("error in (no error)"=w355, "CIF Pcap Subscriber Configuration"=T1 {"Name"="name", "Topic"="topic", "Link Type"=12345, "Backpressure"=TRUE}) -> ("error out"=w343:errorcluster, "CIF Subscriber Refnum"=w353:T5)  [unwired: 8 in]
        n144 = Increment(x=w346) -> (x+1=w345:u8[])
        n145 = while {
          tunnel: w344 -> [w401]
          shift-right: [w409] -> w369
          shift-left: w342 -> [w406]
          shift-right: [w400] -> _
          shift-left: w345 -> [w402]
          tunnel: [w399] -> w361 mode=indexing if=w407
          tunnel: [w401] -> w349
          stop <- w408 stop-if-true
          n146 = call "CIF Publish.vi"("CIF Channel Header Publisher"=T3 {"T0"=0, "T_Out"=0, "T_Tx"=0, "ClockID"=0}, "error in (no error)"=w406, "Timeout ms"=u32 1 ("Timoeut ms"), "Data In"=w402, "Publisher Reference"=w401) -> ("error out"=w405:errorcluster, "Timeout"=w404:bool)  [unwired: 3 in, 2 out]
          n147 = case shown="False" w404 {
            tunnel: w405 -> [w412 w417]
            tunnel: [w412 w417] -> w409
            tunnel: w402 -> [w415 w416]
            tunnel: [w414 w416] -> w400
            tunnel: [TRUE _] -> w407
            frame False {
              n148 = Increment(x=w415) -> (x+1=w414:u8[])
            }
            frame True {
              # "Timeout"
            }
          }
          n149 = Index Array(array=w400) -> (element=w399:u8)  [unwired: 1 in]
          n150 = Equal?(x=w399, y=u8 11) -> (x = y?=w410:bool)
          n151 = Compound Arithmetic op=OR(w410, w409) -> (w408:bool)
        }
        n152 = while {
          shift-right: [w388] -> w364
          shift-left: TRUE -> [w390]
          shift-right: [w378] -> w351
          shift-left: w343 -> [w383]
          tunnel: [w375] -> w367 mode=indexing if=w384
          tunnel: w353 -> [w381]
          tunnel: [w381] -> w352
          tunnel: w346 -> [w377]
          stop <- w385 stop-if-true
          n153 = call "CIF Receive.vi"("error in (no error)"=w383, "Timoeut ms"=u32 2, "Data In"=w377, "Subscriber Reference"=w381) -> ("error out"=w378:errorcluster, "Data Out"=w379:u8[], "Timeout"=w382:bool)  [unwired: 2 in, 3 out]
          n154 = Wait (ms)(milliseconds to wait=u32 10) -> ()  [unwired: 1 out]
          n155 = case shown="True" w382 {
            tunnel: w379 -> [w393 _]
            tunnel: [w394 TRUE] -> w389
            tunnel: [w393 _] -> w376
            tunnel: w377 -> [w392 _]
            frame False {
              n156 = feedback #5(w392) -> (w396:u8[])
              n157 = feedback-in #5(w393) -> ()
              n158 = Increment(x=w396) -> (x+1=w395:u8[])
              n159 = Equal?(x=w395, y=w393) -> (x = y?=w394:bool)
            }
            frame True {
            }
          }
          n160 = Index Array(array=w376) -> (element=w375:u8)  [unwired: 1 in]
          n161 = Compound Arithmetic op=AND(w390, w389) -> (w388:bool)
          n162 = Equal?(x=u8 10, y=w375) -> (x = y?=w386:bool)
          n163 = Compound Arithmetic op=OR(w386, w378) -> (w385:bool)
          n164 = Not(x=w382) -> (.not. x?=w384:bool)
        }
        n165 = Array Size(array=w361) -> (size(s)=w360:i32)
        n166 = call "Destroy CIF Subscriber.vi"("error in (no error)"=w351, "Subscriber Reference"=w352) -> ("error out"=w350:errorcluster)  [unwired: 9 in]
        n167 = Array Size(array=w367) -> (size(s)=w366:i32)
        n168 = Equal?(x=w360, y=10 ("x")) -> (x = y?=w358:bool)
        n169 = Merge Errors(w369, w350) -> (w348:errorcluster)
        n170 = Equal?(x=10, y=w366) -> (x = y?=w363:bool)
        n171 = call "Destroy CIF Publisher.vi"("error in (no error)"=w348, "Publisher Reference"=w349) -> ("error out"=w347:errorcluster)  [unwired: 9 in]
        n172 = Compound Arithmetic op=AND(w358, w364, w363) -> (w362:bool)
        n173 = case shown="False" w362 {
          tunnel: w372 -> [w421 w422]
          tunnel: [w419 w422] -> w371
          tunnel: "Failed delayed writer" -> [w420 _]
          frame False {
            n174 = Concatenate Strings(w421, w420, "\r") -> (w419:string)
          }
          frame True {
          }
        }
      }
    }
  }
  "status" <- w6
  n175 = And Array Elements(Boolean array=w10) -> (logical AND=→"pass":bool)
  n176 = call "Shutdown Iceoryx.vi"("error in (no error)"=w2) -> ("error out"=→"error out":errorcluster)  [unwired: 10 in]
